vi "CSM_Item_Init.vi"(11 "Object":T1) -> ()   [LabVIEW 2017]
uses:
  <resource>/Framework/Providers/API/ItemRef.ctl
  <resource>/Framework/Providers/API/mxLvMenuItem.ctl
panel:
  out "error out":errorcluster
  in  "error in":errorcluster
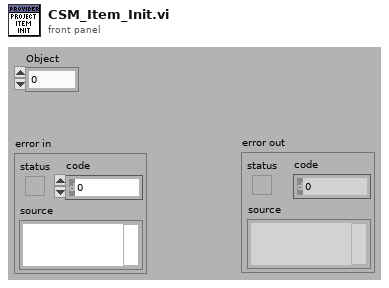
[diagram p1: front panel]
types:
  T1 = typedef "ItemRef.ctl" = u64
  T2 = typedef "mxLvMenuItem.ctl" = cluster{"Menu Name":string, "Description":string, "Icon File Name":path, "Menu Tag":string, "Enabled":bool, "Checked":bool, "Separator":bool, "Batchable":bool, "Weight":i32, "Batch Mode (Ignored if Not Batchable)":enum32{"Show If All Items Support Command", "Show If Any Items Support Command"}, "Menu Location":enum32{"<None>", "Project", "Project / Build Specifications", "Tools", "Tools / Source Control", "Tools / Real-Time Module", "Help"}, "Exclude From Getting Started Window Menu":bool}
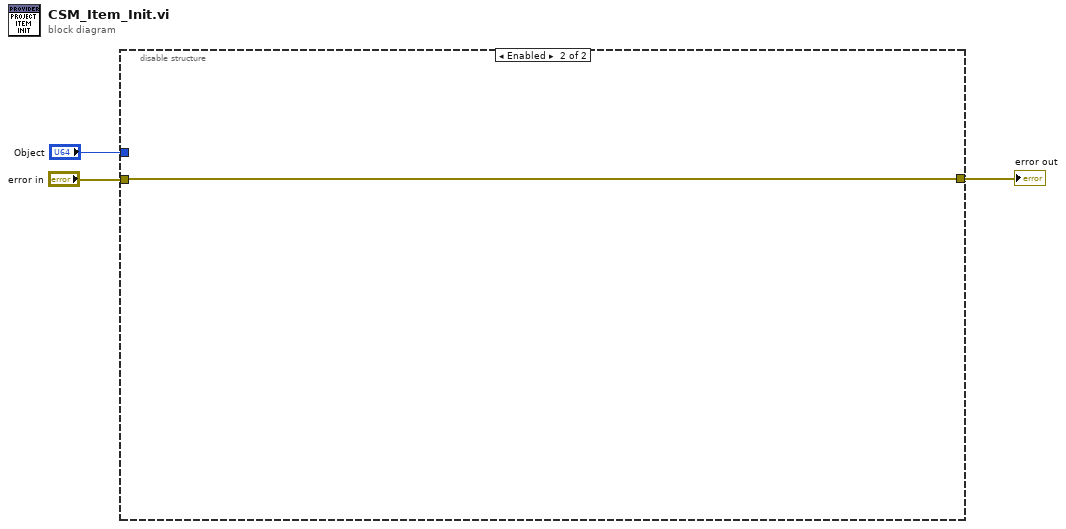
[diagram p0: block diagram]
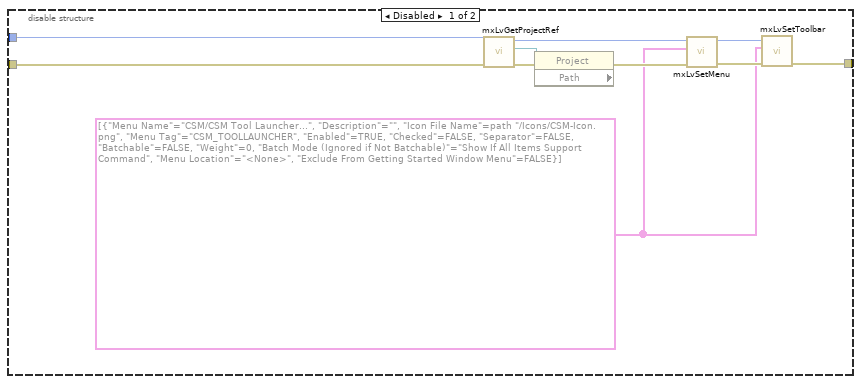
[diagram p2: hidden frame]
diagram:
  n1 = disable-structure shown="Enabled" {
    disable-tunnel: "Object" -> [w7 _]
    disable-tunnel: [w6 w14] -> w2
    disable-tunnel: "error in" -> [w5 w14]
    frame Disabled {
      w4 = T2[] [{"Menu Name"="CSM/CSM Tool Launcher...", "Description"="", "Icon File Name"=path "../Icons/CSM-Icon.png", "Menu Tag"="CSM_TOOLLAUNCHER", "Enabled"=TRUE, "Checked"=FALSE, "Separator"=FALSE, "Batchable"=FALSE, "Weight"=0, "Batch Mode (Ignored if Not Batchable)"=enum."Show If All Items Support Command", "Menu Location"=enum."<None>", "Exclude From Getting Started Window Menu"=FALSE}] ("Array in")
      n2 = call <resource>:"mxLvGetProjectRef.vi"("error in"=w5, "Item"=w7) -> ("error out"=w11:errorcluster, "Project Refnum"=w10:refnum<vi>, "Item"=w9:T1)  [unwired: 7 in]
      n3 = property class="Project" props=["Path"](reference=w10, error in=w11) -> (error out=w8:errorcluster)  [unwired: 2 out]
      n4 = call <resource>:"mxLvSetMenu.vi"("error in"=w8, "Menu Items"=w4, "Item"=w9) -> ("error out"=w12:errorcluster, "Item"=w13:T1)  [unwired: 7 out]
      n5 = call <resource>:"mxLvSetToolbar.vi"("error in"=w12, "Toolbar Items"=w4, "Item"=w13) -> ("error out"=w6:errorcluster)  [unwired: 7 in, 1 out]
    }
    frame Enabled {
    }
  }
  "error out" <- w2
